vi "NR set HO Center Channel.vi"(8 "error in (no error)":errorcluster caption="에러 입력(에러 없음)", 10 "Center Channel Number":u32, 11 "Instrument Manager 입력":refnum<class "Instrument Manager.lvclass">) -> (0 "error out":errorcluster caption="에러 출력", 3 "Instrument Manager 출력":refnum<class "Instrument Manager.lvclass">)   [LabVIEW 2023, in "Instrument Manager.lvclass"]
uses:
  Instrument Manager.lvclass
  Instrument Manager.lvclass/Instrument Manager.ctl
  Module/ANRITSU Call Box/Interface Class/Anritsu Call Box.lvclass
  Module/ANRITSU Call Box/Type Definition/Uplink Downlink Enum.ctl
  Module/ANRITSU Call Box/ANRITSU Call Box.lvlib
  Module/ANRITSU Call Box/Type Definition/NR Center Channel Arguments.ctl
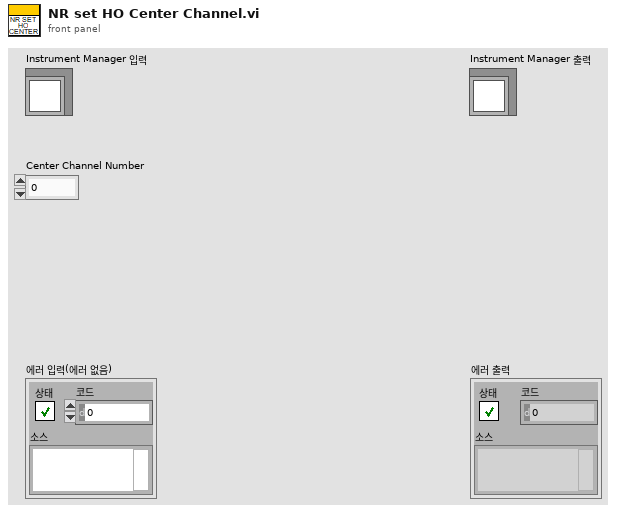
[diagram p1: front panel]
types:
  T1 = typedef "ANRITSU Call Box.lvlib/NR Center Channel Arguments.ctl" = cluster{"Center Channel Number":u32, "Selected CC":enum16{"PCC", "SCC", "FR2_PCC", "FR2_SCC"}, "SCC or FR2_SCC Index":u32}
  T2 = typedef "ANRITSU Call Box.lvlib/Uplink Downlink Enum.ctl" = enum16{"Uplink", "Downlink"}
  T3 = cluster{"Anritsu Call Box":refnum<class "Anritsu Call Box.lvclass">, "Spectrum Analyzer":refnum<class "Interface_Spectrum.lvclass">, "RF Switch Box":refnum<class "RF Filter Box.lvclass">, "Turn Table":refnum<class "Interface - Turn Table.lvclass">, "Mast":refnum<class "Interface - Mast.lvclass">, "3D Controller":refnum<class "Interface_3D Controller.lvclass">}
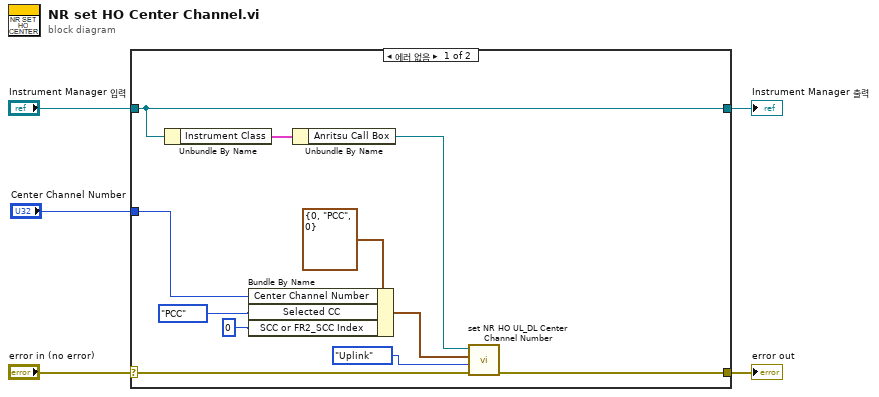
[diagram p0: block diagram]
diagram:
  n1 = case shown="에러 없음" "error in (no error)" {
    selector: "error in (no error)" -> [w16 w18]
    tunnel: [w15 w18] -> w4
    tunnel: [w14 w17] -> w2
    tunnel: "Instrument Manager 입력" -> [w14 w17]
    tunnel: "Center Channel Number" -> [w9 _]
    frame No Error {
      n2 = Unbundle By Name(w14) -> ("Instrument Class"=w13:T3)
      n3 = Bundle By Name(cluster=T1 {"Center Channel Number"=0, "Selected CC"=enum."PCC", "SCC or FR2_SCC Index"=0} ("Center Channel Argements"), "Center Channel Number"=w9, "Selected CC"=enum16{"PCC", "SCC", "FR2_PCC", "FR2_SCC"}."PCC", "SCC or FR2_SCC Index"=u32 0) -> (w8:T1)
      n4 = Unbundle By Name(w13) -> ("Anritsu Call Box"=w12:refnum<class "Anritsu Call Box.lvclass">)
      n5 = call-dynamic "set NR HO UL_DL Center Channel Number.vi"("error in (no error)"=w16, "Direction"=Uplink_Downlink_Enum."Uplink", "Center Channel Argements"=w8, "Anritsu Call Box 입력"=w12) -> ("error out"=w15:errorcluster)  [unwired: 6 in, 1 out]
    }
    frame Error {
    }
  }
  "error out" <- w4
  "Instrument Manager 출력" <- w2
